vi "FTCU LS_G100Test.vi"() -> ()   [LabVIEW 2019]
uses:
  <vilib>/NI/Modbus Library/API/Wrapper/Create Serial Master.vi
  <vilib>/NI/Modbus Library/API/Master/Modbus Master.lvclass
  <vilib>/NI/Modbus Library/API/Wrapper/API Main.lvlib
panel:
  out "input reg values hex":u16[](array[numeric]) format="%04x"
  out "input reg values":u16[](array[numeric])
  in  "no input reg":u16
  in  "address input":u16=896 format="%04x"
  in  "number of inputs 2":u16=2
  out "element 1":u16 format="%016b"
  out "element 0":u16 format="%016b"
  out "(hi.lo)":sgl format="%.2f"
  in  "register to write":u16=50
  out "read values":u16[](array[numeric])
  in  "read count":u16=1
  in  "read starting address":u16=302 format="%04d"
  out "error out":errorcluster
  out "FTCU Input Reg Value":u16[](array[numeric])
  in  "FTCU Hold Reg Addr":u16=302 format="%04d"
  in  "FTCU Input Reg Addr":u16=8 format="%04d"
  in  "stop":bool
  in  "frequency":u16 caption="frequency, 0.01 Hz"
  in  "address":u16=896 format="%04x"
  in  "number of inputs":u16=1
  in  "read holdin address":u16=19 format="%04x"
  out "holding reg values":u16[](array[numeric])
  # "G100"
  # "Holding read"
  # "2 Hz to minimum"
  # "0h0380 - adres zadawania prêdkoœci\ntab 7.6.2, str. 236"
  # "FTCU"
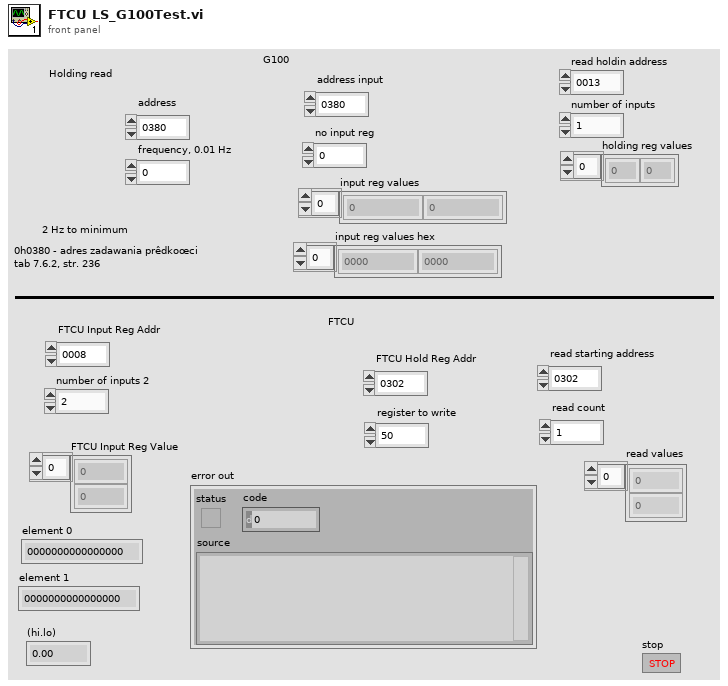
[diagram p1: front panel]
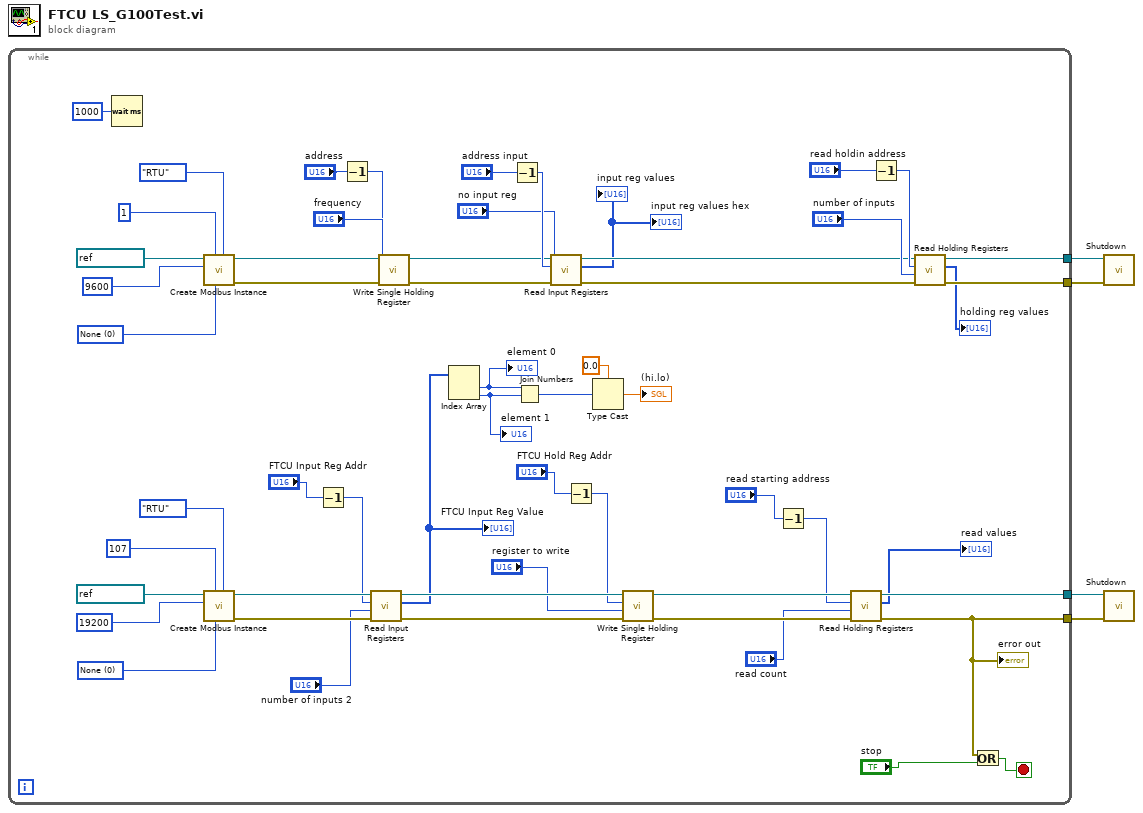
[diagram p0: block diagram]
diagram:
  n1 = while {
    tunnel: [w54] -> w4
    tunnel: [w53] -> w3
    tunnel: [w36] -> w1
    tunnel: [w34] -> w2
    stop <- w39 stop-if-true
    w45 = u16 0 items=["None", "Odd", "Even", "Mark", "Space"] ("parity (even)")
    w58 = u16 0 items=["None", "Odd", "Even", "Mark", "Space"] ("parity (even)")
    n2 = Wait (ms)(milliseconds to wait=u32 1000) -> ()  [unwired: 1 out]
    n3 = call-poly <vilib>:"Create Modbus Instance.vi"("serial type"=enum16{"RTU", "ASCII"}."RTU", "parity (even)"=w58, "unit ID"=u8 1, "baud rate"=u32 9600, "VISA resource name"=refnum<visa-resource-name> "COM21") -> ("error out"=w51:errorcluster, "serial master instance"=w50:refnum<class "Modbus Master.lvclass">)  [unwired: 5 in]
    n4 = call-poly <vilib>:"Create Modbus Instance.vi"("serial type"=enum16{"RTU", "ASCII"}."RTU", "parity (even)"=w45, "unit ID"=u8 107, "baud rate"=u32 19200, "VISA resource name"=refnum<visa-resource-name> "COM22") -> ("error out"=w41:errorcluster, "serial master instance"=w42:refnum<class "Modbus Master.lvclass">)  [unwired: 5 in]
    n5 = Decrement(x="FTCU Input Reg Addr") -> (x-1=w26:u16)
    n6 = Decrement(x="address") -> (x-1=w15:u16)
    n7 = call-dynamic "Read Input Registers.vi"("error in"=w41, "number of inputs"="number of inputs 2", "starting address"=w26, "Modbus master in"=w42) -> ("error out"=w27:errorcluster, "register values"=w22:u16[], "Modbus master out"=w28:refnum<class "Modbus Master.lvclass">)  [unwired: 5 in]
    "FTCU Input Reg Value" <- w22
    n8 = call-dynamic "Write Single Holding Register.vi"("error in"=w51, "register to write"="frequency", "address"=w15, "Modbus master in"=w50) -> ("error out"=w10:errorcluster, "Modbus master out"=w11:refnum<class "Modbus Master.lvclass">)  [unwired: 6 in]
    n9 = Index Array(array=w22) -> (element #1=w21:u16, element #2=w20:u16)  [unwired: 2 in]
    "element 0" <- w21
    "element 1" <- w20
    n10 = Decrement(x="address input") -> (x-1=w12:u16)
    n11 = Join Numbers(hi=w21, lo=w20) -> ((hi.lo)=w19:u32)
    n12 = call-dynamic "Read Input Registers.vi"("error in"=w10, "number of inputs"="no input reg", "starting address"=w12, "Modbus master in"=w11) -> ("error out"=w8:errorcluster, "register values"=→"input reg values" →"input reg values hex":u16[], "Modbus master out"=w9:refnum<class "Modbus Master.lvclass">)  [unwired: 5 in]
    n13 = Decrement(x="FTCU Hold Reg Addr") -> (x-1=w24:u16)
    n14 = Type Cast(type=sgl 0.0, x=w19) -> (*(type *) &x=→"(hi.lo)":sgl)
    n15 = call-dynamic "Write Single Holding Register.vi"("error in"=w27, "register to write"="register to write", "address"=w24, "Modbus master in"=w28) -> ("error out"=w35:errorcluster, "Modbus master out"=w37:refnum<class "Modbus Master.lvclass">)  [unwired: 6 in]
    n16 = Decrement(x="read starting address") -> (x-1=w30:u16)
    n17 = call-dynamic "Read Holding Registers.vi"("error in"=w35, "number of inputs"="read count", "starting address"=w30, "Modbus master in"=w37) -> ("error out"=w34:errorcluster, "register values"=→"read values":u16[], "Modbus master out"=w36:refnum<class "Modbus Master.lvclass">)  [unwired: 5 in]
    "error out" <- w34
    n18 = Decrement(x="read holdin address") -> (x-1=w13:u16)
    n19 = call-dynamic "Read Holding Registers.vi"("error in"=w8, "number of inputs"="number of inputs", "starting address"=w13, "Modbus master in"=w9) -> ("error out"=w54:errorcluster, "register values"=→"holding reg values":u16[], "Modbus master out"=w53:refnum<class "Modbus Master.lvclass">)  [unwired: 5 in]
    n20 = Or(x=w34, y="stop") -> (x .or. y?=w39:bool)
  }
  n21 = call-dynamic "Shutdown.vi"("error in"=w4, "Modbus master in"=w3) -> ()  [unwired: 9 in, 1 out]
  n22 = call-dynamic "Shutdown.vi"("error in"=w2, "Modbus master in"=w1) -> ()  [unwired: 9 in, 1 out]
